vi "Lire_fichier_profil EPC3000.vi"(2 "error in (no error)":errorcluster caption="entrée d'erreur (pas d'erreur)", 3 "Chemin du fichier profil":path caption="chemin du fichier profil") -> (0 "error out":errorcluster caption="entrée d'erreur (pas d'erreur)", 1 "Config + programmes":T1 {"config"."value" format="%#.1f"})   [LabVIEW 2022 SP3]
uses:
  <vilib>/Utility/config.llb/Read Key (Double).vi
  <vilib>/Utility/config.llb/NI_LVConfig.lvlib
panel:
  out "Programme 10":cluster{string, dbl}[][](array[cluster]) {"?" format="%#.1f"}
  out "Programme 9":cluster{string, dbl}[][](array[cluster]) {"?" format="%#.1f"}
  out "Programme 8":cluster{string, dbl}[][](array[cluster]) {"?" format="%#.1f"}
  out "Programme 7":cluster{string, dbl}[][](array[cluster]) {"?" format="%#.1f"}
  out "Programme 6":cluster{string, dbl}[][](array[cluster]) {"?" format="%#.1f"}
  out "Programme 5":cluster{string, dbl}[][](array[cluster]) {"?" format="%#.1f"}
  out "Chemin du fichier en sortie":path caption="chemin du fichier"
  out "Programme 4":cluster{string, dbl}[][](array[cluster]) {"?" format="%#.1f"}
  out "Programme 3":cluster{string, dbl}[][](array[cluster]) {"?" format="%#.1f"}
  out "Programme 2":cluster{string, dbl}[][](array[cluster]) {"?" format="%#.1f"}
  out "Programme 1":cluster{string, dbl}[][](array[cluster]) {"?" format="%#.1f"}
  out "Configuration":cluster{"key":string, "value":dbl}[](array[cluster]) {"value" format="%#.1f"}
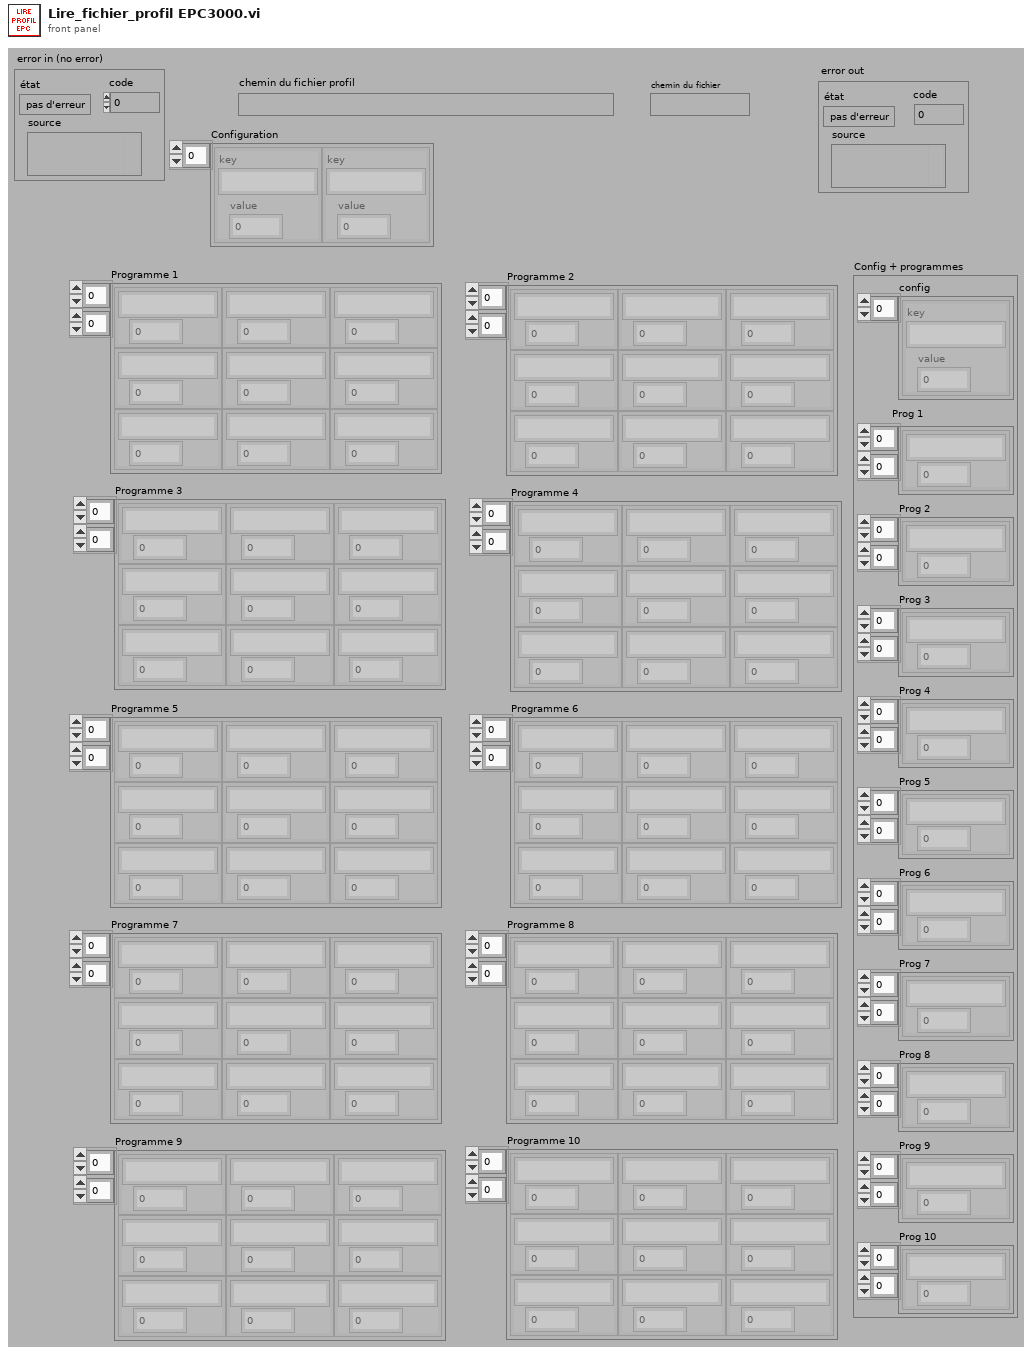
[diagram p1: front panel]
types:
  T1 = cluster{"config":cluster{"key":string, "value":dbl}[], "Prog 1":cluster{string, dbl}[][], "Prog 2":cluster{string, dbl}[][], "Prog 3":cluster{string, dbl}[][], "Prog 4":cluster{string, dbl}[][], "Prog 5":cluster{string, dbl}[][], "Prog 6":cluster{string, dbl}[][], "Prog 7":cluster{string, dbl}[][], "Prog 8":cluster{string, dbl}[][], "Prog 9":cluster{string, dbl}[][], "Prog 10":cluster{string, dbl}[][]}
  T2 = typedef "NI_LVConfig.lvlib/Config Data RefNum.ctl" = refnum<k1>
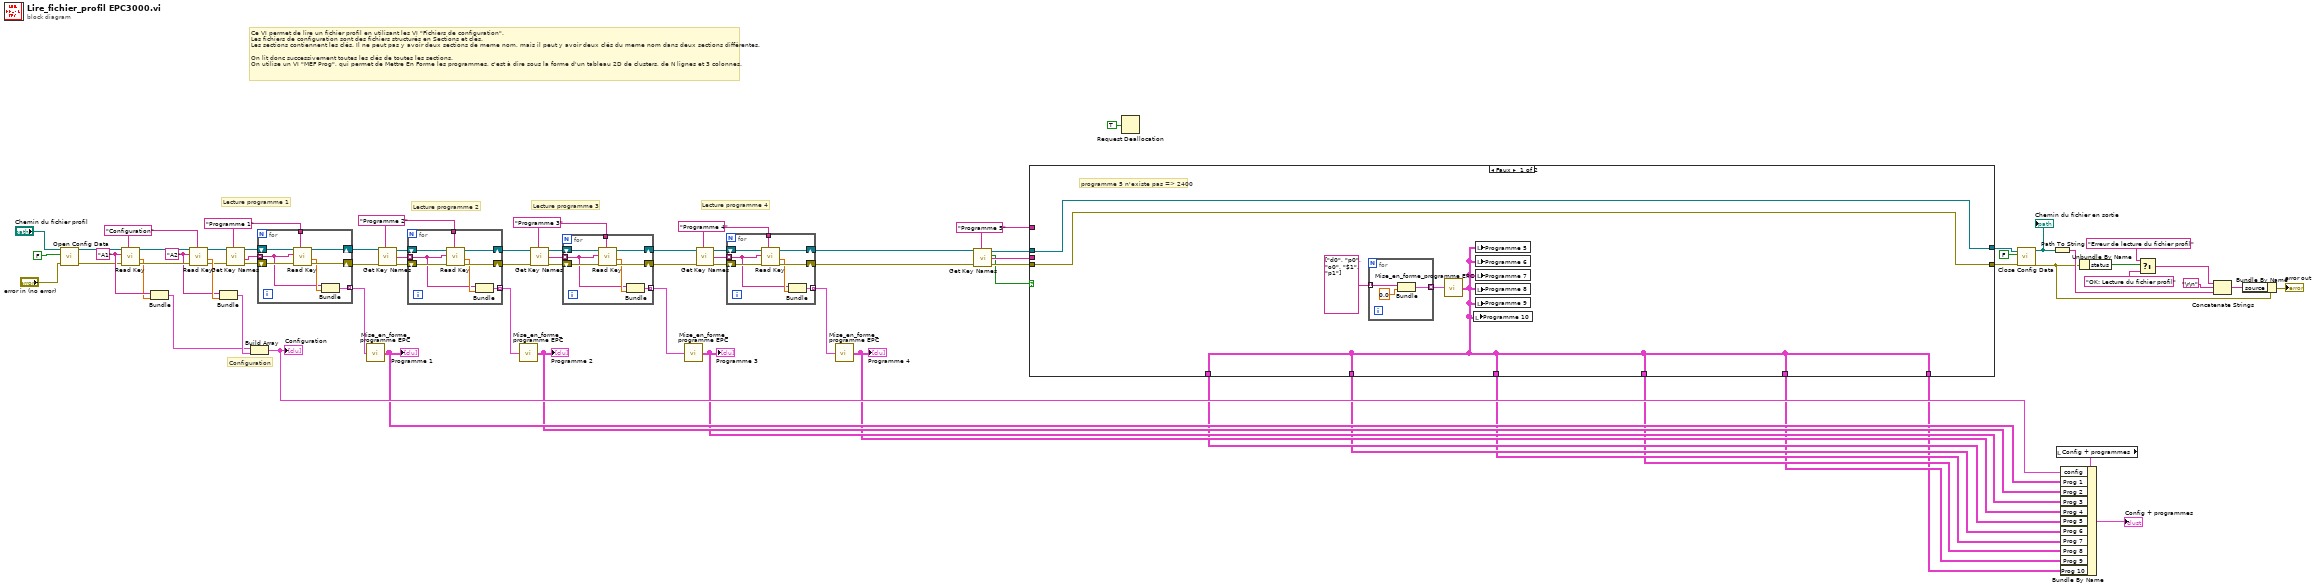
[diagram p0: block diagram]
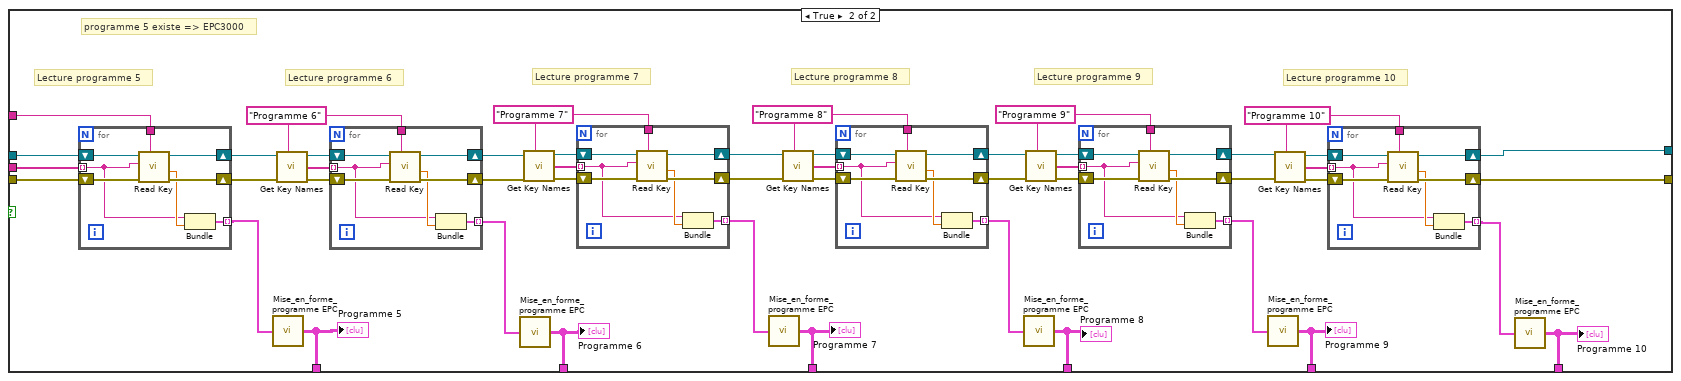
[diagram p2: hidden frame]
diagram:
  w24 = "Programme 5"
  w45 = "Programme 4"
  w51 = "Programme 3"
  w59 = "Programme 2"
  w67 = "Programme 1"
  w71 = "A1" ("key")
  w72 = "A2" ("key")
  w74 = "Configuration" ("section")
  # "Ce VI permet de lire un fichier profil en utilisant les VI \"Fichiers de configuration\".\nLes fichiers de configuration sont des fichiers structurés en Sections et clés. \nLes sections contiennent les clés. Il ne peut pas y avoir deux sections de meme nom, mais il peut y avoir deux clés du meme nom dans deux sections différentes.\n\nOn lit donc successivement toutes les clés de toutes les sections.\nOn utilise un VI \"MEF Prog\", qui permet de Mettre En Forme les programmes, c'est à dire sous la forme d'un tableau 2D de clusters, de N lignes et 3 colonnes."
  # "Lecture programme 4"
  # "Lecture programme 3"
  # "Lecture programme 2"
  # "Lecture programme 1"
  # "Configuration"
  n1 = call <vilib>:"Open Config Data.vi"("error in (no error)"="error in (no error)", "create file if necessary (T)"=FALSE ("create file if necessary? (T)"), "configuration file path"="Chemin du fichier profil") -> ("error out"=w34:errorcluster, "refnum"=w35:T2)  [unwired: 6 in, 1 out]
  n2 = call-poly <vilib>:"Read Key.vi"("section"=w74, "error in (no error)"=w34, "key"=w71, "refnum"=w35) -> ("error out"=w76:errorcluster, "value"=w70:dbl, "refnum out"=w75:T2)  [unwired: 4 in, 1 out]
  n3 = Bundle("key"=w71, "value"=w70) -> (w68:cluster{"key":string, "value":dbl})  [unwired: 1 in]
  n4 = call-poly <vilib>:"Read Key.vi"("section"=w74, "error in (no error)"=w76, "key"=w72, "refnum"=w75) -> ("error out"=w63:errorcluster, "value"=w73:dbl, "refnum out"=w64:T2)  [unwired: 4 in, 1 out]
  n5 = Bundle("key"=w72, "value"=w73) -> (w69:cluster{"key":string, "value":dbl})  [unwired: 1 in]
  n6 = call <vilib>:"Get Key Names.vi"("section"=w67, "error in (no error)"=w63, "refnum"=w64) -> ("error out"=w66:errorcluster, "key names"=w38:string[], "refnum out"=w65:T2)  [unwired: 5 in, 1 out]
  n7 = Build Array(w68, w69) -> (w15:cluster{"key":string, "value":dbl}[])
  "Configuration" <- w15
  n8 = for {
    shift-right: [w82] -> w58
    shift-left: w65 -> [w84]
    shift-right: [w81] -> w57
    shift-left: w66 -> [w83]
    tunnel: w67 -> [w80]
    tunnel: w38 -> [w77] mode=indexing
    tunnel: [w78] -> w39 mode=indexing
    n9 = call-poly <vilib>:"Read Key.vi"("section"=w80, "error in (no error)"=w83, "key"=w77, "refnum"=w84) -> ("error out"=w81:errorcluster, "value"=w79:dbl, "refnum out"=w82:T2)  [unwired: 4 in, 1 out]
    n10 = Bundle("String"=w77, "value"=w79) -> (w78:cluster{"String":string, "value":dbl})  [unwired: 1 in]
  }
  n11 = call "Mise_en_forme_programme EPC.vi"("Programme en entrée"=w39) -> ("Programme en sortie"=w13:cluster{string, dbl}[][])
  "Programme 1" <- w13
  n12 = call <vilib>:"Get Key Names.vi"("section"=w59, "error in (no error)"=w57, "refnum"=w58) -> ("error out"=w61:errorcluster, "key names"=w60:string[], "refnum out"=w62:T2)  [unwired: 5 in, 1 out]
  n13 = for {
    shift-right: [w90] -> w52
    shift-left: w62 -> [w92]
    shift-right: [w89] -> w53
    shift-left: w61 -> [w91]
    tunnel: w59 -> [w88]
    tunnel: w60 -> [w86] mode=indexing
    tunnel: [w85] -> w43 mode=indexing
    n14 = call-poly <vilib>:"Read Key.vi"("section"=w88, "error in (no error)"=w91, "key"=w86, "refnum"=w92) -> ("error out"=w89:errorcluster, "value"=w87:dbl, "refnum out"=w90:T2)  [unwired: 4 in, 1 out]
    n15 = Bundle("String"=w86, "value"=w87) -> (w85:cluster{"String":string, "value":dbl})  [unwired: 1 in]
  }
  n16 = call "Mise_en_forme_programme EPC.vi"("Programme en entrée"=w43) -> ("Programme en sortie"=w12:cluster{string, dbl}[][])
  "Programme 2" <- w12
  n17 = call <vilib>:"Get Key Names.vi"("section"=w51, "error in (no error)"=w53, "refnum"=w52) -> ("error out"=w55:errorcluster, "key names"=w56:string[], "refnum out"=w54:T2)  [unwired: 5 in, 1 out]
  n18 = for {
    shift-right: [w98] -> w47
    shift-left: w54 -> [w100]
    shift-right: [w97] -> w46
    shift-left: w55 -> [w99]
    tunnel: w51 -> [w96]
    tunnel: w56 -> [w94] mode=indexing
    tunnel: [w93] -> w42 mode=indexing
    n19 = call-poly <vilib>:"Read Key.vi"("section"=w96, "error in (no error)"=w99, "key"=w94, "refnum"=w100) -> ("error out"=w97:errorcluster, "value"=w95:dbl, "refnum out"=w98:T2)  [unwired: 4 in, 1 out]
    n20 = Bundle("String"=w94, "value"=w95) -> (w93:cluster{"String":string, "value":dbl})  [unwired: 1 in]
  }
  n21 = call "Mise_en_forme_programme EPC.vi"("Programme en entrée"=w42) -> ("Programme en sortie"=w11:cluster{string, dbl}[][])
  "Programme 3" <- w11
  n22 = call <vilib>:"Get Key Names.vi"("section"=w45, "error in (no error)"=w46, "refnum"=w47) -> ("error out"=w49:errorcluster, "key names"=w48:string[], "refnum out"=w50:T2)  [unwired: 5 in, 1 out]
  n23 = for {
    shift-right: [w106] -> w20
    shift-left: w50 -> [w108]
    shift-right: [w105] -> w19
    shift-left: w49 -> [w107]
    tunnel: w45 -> [w104]
    tunnel: w48 -> [w102] mode=indexing
    tunnel: [w101] -> w41 mode=indexing
    n24 = call-poly <vilib>:"Read Key.vi"("section"=w104, "error in (no error)"=w107, "key"=w102, "refnum"=w108) -> ("error out"=w105:errorcluster, "value"=w103:dbl, "refnum out"=w106:T2)  [unwired: 4 in, 1 out]
    n25 = Bundle("String"=w102, "value"=w103) -> (w101:cluster{"String":string, "value":dbl})  [unwired: 1 in]
  }
  n26 = call "Mise_en_forme_programme EPC.vi"("Programme en entrée"=w41) -> ("Programme en sortie"=w10:cluster{string, dbl}[][])
  "Programme 4" <- w10
  n27 = call <vilib>:"Get Key Names.vi"("section"=w24, "error in (no error)"=w19, "refnum"=w20) -> ("error out"=w22:errorcluster, "key names"=w23:string[], "section exists?"=w3:bool, "refnum out"=w21:T2)  [unwired: 5 in]
  n28 = case shown="Faux" w3 {
    tunnel: w24 -> [_ w164]
    tunnel: w23 -> [_ w163]
    tunnel: w22 -> [w112 w162]
    tunnel: w21 -> [w113 w161]
    tunnel: [w113 w130] -> w18
    tunnel: [w112 w129] -> w17
    tunnel: [w109 w122] -> w9
    tunnel: [w109 w121] -> w8
    tunnel: [w109 w120] -> w7
    tunnel: [w109 w119] -> w6
    tunnel: [w109 w118] -> w5
    tunnel: [w109 w117] -> w4
    frame False {
      # "programme 5 n'existe pas => 2400"
      n29 = for {
        tunnel: string[] ["d0", "p0", "o0", "$1", "p1"] -> [w115] mode=indexing
        tunnel: [w114] -> w111 mode=indexing
        n30 = Bundle(w115, 0.0) -> (w114:cluster{string, dbl})  [unwired: 1 in]
      }
      n31 = call "Mise_en_forme_programme EPC.vi"("Programme en entrée"=w111) -> ("Programme en sortie"=w109:cluster{string, dbl}[][])
      n32 = local write "Programme 10"(w109) -> ()
      n33 = local write "Programme 5"(w109) -> ()
      n34 = local write "Programme 6"(w109) -> ()
      n35 = local write "Programme 7"(w109) -> ()
      n36 = local write "Programme 8"(w109) -> ()
      n37 = local write "Programme 9"(w109) -> ()
    }
    frame True {
      w141 = "Programme 10"
      w148 = "Programme 9"
      w149 = "Programme 8"
      w156 = "Programme 7"
      w157 = "Programme 6"
      # "programme 5 existe => EPC3000"
      # "Lecture programme 10"
      # "Lecture programme 9"
      # "Lecture programme 8"
      # "Lecture programme 7"
      # "Lecture programme 6"
      # "Lecture programme 5"
      n38 = for {
        shift-right: [w210] -> w140
        shift-left: w161 -> [w212]
        shift-right: [w209] -> w139
        shift-left: w162 -> [w211]
        tunnel: w164 -> [w208]
        tunnel: w163 -> [w206] mode=indexing
        tunnel: [w205] -> w128 mode=indexing
        n39 = call-poly <vilib>:"Read Key.vi"("section"=w208, "error in (no error)"=w211, "key"=w206, "refnum"=w212) -> ("error out"=w209:errorcluster, "value"=w207:dbl, "refnum out"=w210:T2)  [unwired: 4 in, 1 out]
        n40 = Bundle("String"=w206, "value"=w207) -> (w205:cluster{"String":string, "value":dbl})  [unwired: 1 in]
      }
      n41 = call "Mise_en_forme_programme EPC.vi"("Programme en entrée"=w128) -> ("Programme en sortie"=w122:cluster{string, dbl}[][])
      "Programme 5" <- w122
      n42 = call <vilib>:"Get Key Names.vi"("section"=w157, "error in (no error)"=w139, "refnum"=w140) -> ("error out"=w159:errorcluster, "key names"=w158:string[], "refnum out"=w160:T2)  [unwired: 5 in, 1 out]
      n43 = for {
        shift-right: [w202] -> w138
        shift-left: w160 -> [w204]
        shift-right: [w201] -> w137
        shift-left: w159 -> [w203]
        tunnel: w157 -> [w200]
        tunnel: w158 -> [w198] mode=indexing
        tunnel: [w197] -> w127 mode=indexing
        n44 = call-poly <vilib>:"Read Key.vi"("section"=w200, "error in (no error)"=w203, "key"=w198, "refnum"=w204) -> ("error out"=w201:errorcluster, "value"=w199:dbl, "refnum out"=w202:T2)  [unwired: 4 in, 1 out]
        n45 = Bundle("String"=w198, "value"=w199) -> (w197:cluster{"String":string, "value":dbl})  [unwired: 1 in]
      }
      n46 = call "Mise_en_forme_programme EPC.vi"("Programme en entrée"=w127) -> ("Programme en sortie"=w121:cluster{string, dbl}[][])
      "Programme 6" <- w121
      n47 = call <vilib>:"Get Key Names.vi"("section"=w156, "error in (no error)"=w137, "refnum"=w138) -> ("error out"=w154:errorcluster, "key names"=w155:string[], "refnum out"=w153:T2)  [unwired: 5 in, 1 out]
      n48 = for {
        shift-right: [w194] -> w136
        shift-left: w153 -> [w196]
        shift-right: [w193] -> w135
        shift-left: w154 -> [w195]
        tunnel: w156 -> [w192]
        tunnel: w155 -> [w190] mode=indexing
        tunnel: [w189] -> w126 mode=indexing
        n49 = call-poly <vilib>:"Read Key.vi"("section"=w192, "error in (no error)"=w195, "key"=w190, "refnum"=w196) -> ("error out"=w193:errorcluster, "value"=w191:dbl, "refnum out"=w194:T2)  [unwired: 4 in, 1 out]
        n50 = Bundle("String"=w190, "value"=w191) -> (w189:cluster{"String":string, "value":dbl})  [unwired: 1 in]
      }
      n51 = call "Mise_en_forme_programme EPC.vi"("Programme en entrée"=w126) -> ("Programme en sortie"=w120:cluster{string, dbl}[][])
      "Programme 7" <- w120
      n52 = call <vilib>:"Get Key Names.vi"("section"=w149, "error in (no error)"=w135, "refnum"=w136) -> ("error out"=w151:errorcluster, "key names"=w150:string[], "refnum out"=w152:T2)  [unwired: 5 in, 1 out]
      n53 = for {
        shift-right: [w186] -> w134
        shift-left: w152 -> [w188]
        shift-right: [w185] -> w133
        shift-left: w151 -> [w187]
        tunnel: w149 -> [w184]
        tunnel: w150 -> [w182] mode=indexing
        tunnel: [w181] -> w125 mode=indexing
        n54 = call-poly <vilib>:"Read Key.vi"("section"=w184, "error in (no error)"=w187, "key"=w182, "refnum"=w188) -> ("error out"=w185:errorcluster, "value"=w183:dbl, "refnum out"=w186:T2)  [unwired: 4 in, 1 out]
        n55 = Bundle("String"=w182, "value"=w183) -> (w181:cluster{"String":string, "value":dbl})  [unwired: 1 in]
      }
      n56 = call "Mise_en_forme_programme EPC.vi"("Programme en entrée"=w125) -> ("Programme en sortie"=w119:cluster{string, dbl}[][])
      "Programme 8" <- w119
      n57 = call <vilib>:"Get Key Names.vi"("section"=w148, "error in (no error)"=w133, "refnum"=w134) -> ("error out"=w146:errorcluster, "key names"=w147:string[], "refnum out"=w145:T2)  [unwired: 5 in, 1 out]
      n58 = for {
        shift-right: [w178] -> w132
        shift-left: w145 -> [w180]
        shift-right: [w177] -> w131
        shift-left: w146 -> [w179]
        tunnel: w148 -> [w176]
        tunnel: w147 -> [w174] mode=indexing
        tunnel: [w173] -> w124 mode=indexing
        n59 = call-poly <vilib>:"Read Key.vi"("section"=w176, "error in (no error)"=w179, "key"=w174, "refnum"=w180) -> ("error out"=w177:errorcluster, "value"=w175:dbl, "refnum out"=w178:T2)  [unwired: 4 in, 1 out]
        n60 = Bundle("String"=w174, "value"=w175) -> (w173:cluster{"String":string, "value":dbl})  [unwired: 1 in]
      }
      n61 = call "Mise_en_forme_programme EPC.vi"("Programme en entrée"=w124) -> ("Programme en sortie"=w118:cluster{string, dbl}[][])
      "Programme 9" <- w118
      n62 = call <vilib>:"Get Key Names.vi"("section"=w141, "error in (no error)"=w131, "refnum"=w132) -> ("error out"=w143:errorcluster, "key names"=w142:string[], "refnum out"=w144:T2)  [unwired: 5 in, 1 out]
      n63 = for {
        shift-right: [w170] -> w130
        shift-left: w144 -> [w172]
        shift-right: [w169] -> w129
        shift-left: w143 -> [w171]
        tunnel: w141 -> [w168]
        tunnel: w142 -> [w166] mode=indexing
        tunnel: [w165] -> w123 mode=indexing
        n64 = call-poly <vilib>:"Read Key.vi"("section"=w168, "error in (no error)"=w171, "key"=w166, "refnum"=w172) -> ("error out"=w169:errorcluster, "value"=w167:dbl, "refnum out"=w170:T2)  [unwired: 4 in, 1 out]
        n65 = Bundle("String"=w166, "value"=w167) -> (w165:cluster{"String":string, "value":dbl})  [unwired: 1 in]
      }
      n66 = call "Mise_en_forme_programme EPC.vi"("Programme en entrée"=w123) -> ("Programme en sortie"=w117:cluster{string, dbl}[][])
      "Programme 10" <- w117
    }
  }
  n67 = Request Deallocation(TRUE ("flag")) -> ()
  n68 = call <vilib>:"Close Config Data.vi"("error in (no error)"=w17, "write file if changed (T)"=FALSE ("write configuration file? (T)"), "refnum"=w18) -> ("error out"=w26:errorcluster, "file path"=w40:path)  [unwired: 7 in]
  "Chemin du fichier en sortie" <- w40
  n69 = Path To String(path=w40) -> (string=w28:string)
  n70 = local read "Config + programmes"() -> (w16:T1)
  n71 = Bundle By Name(cluster=w16, "config"=w15, "Prog 1"=w13, "Prog 2"=w12, "Prog 3"=w11, "Prog 4"=w10, "Prog 5"=w9, "Prog 6"=w8, "Prog 7"=w7, "Prog 8"=w6, "Prog 9"=w5, "Prog 10"=w4) -> (→"Config + programmes":T1)
  n72 = Unbundle By Name(w26) -> ("status"=w32:bool)
  n73 = Select(t="Erreur de lecture du fichier profil", s=w32, f="OK: Lecture du fichier profil") -> (s? t:f=w29:string)
  n74 = Concatenate Strings(w29, "\r\n", w28) -> (w25:string)
  n75 = Bundle By Name(cluster=w26, "source"=w25) -> (→"error out":errorcluster)
